vi "Lookup ETag.vi"(8 "error in (no error)":errorcluster, 10 "ETag":string, 11 "Caching in":refnum<class "Caching.lvclass">) -> (0 "error out":errorcluster, 1 "From Cache?":bool, 2 "Response":refnum<class "Response.lvclass">, 3 "Caching out":refnum<class "Caching.lvclass">)   [LabVIEW 2020, in "HTTP Server.lvlib" / "Caching.lvclass"]
uses:
  Caching.lvclass
  lv-http-util/HTTP Utils/Response/Response.lvclass
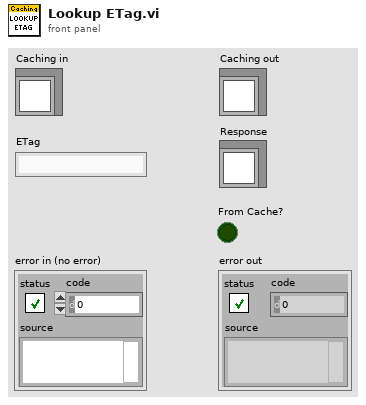
[diagram p1: front panel]
types:
  T1 = typedef "HTTP Server.lvlib/Caching.lvclass/Cache Item.ctl" = cluster{"ID":string, "File":bool, "Path":path, "Value":string, "Created":timestamp, "Expires":timestamp}
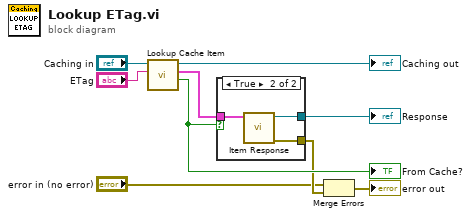
[diagram p0: block diagram]
diagram:
  n1 = call "Lookup Cache Item.vi"("ID"="ETag", "Caching in"="Caching in") -> ("Found?"=w4:bool, "Cache Item"=w7:T1, "Caching out"=→"Caching out":refnum<class "Caching.lvclass">)  [unwired: 6 in, 1 out]
  "From Cache?" <- w4
  n2 = case shown="True" w4 {
    tunnel: w7 -> [_ w12]
    tunnel: [_ w11] -> w5
    tunnel: [_ w10] -> w3
    frame False {
    }
    frame True {
      n3 = call "Item Response.vi"("Cache Item"=w12) -> ("error out"=w10:errorcluster, "Response"=w11:refnum<class "Response.lvclass">)  [unwired: 9 in]
    }
  }
  "Response" <- w5
  n4 = Merge Errors("error in (no error)", w3) -> (→"error out":errorcluster)
